vi "dfreq.vi"() -> ()   [LabVIEW 2019]
uses:
  <vilib>/DAQmx/read.llb/DAQmx Read (Counter DBL 1Chan 1Samp).vi
  <vilib>/DAQmx/create/channels.llb/DAQmx Create Channel (CO-Pulse Generation-Ticks).vi
  <vilib>/DAQmx/create/channels.llb/DAQmx Create Channel (CI-Frequency).vi
  <vilib>/DAQmx/configure/timing.llb/DAQmx Timing (Implicit).vi
  <vilib>/DAQmx/configure/trigger.llb/DAQmx Start Trigger (Digital Edge).vi
  <vilib>/DAQmx/miscellaneous.llb/DAQmx Fill In Error Info.vi
  <resource>/objmgr/daqmx.rc
panel:
  out "highest harmonic":i32
  out "counter":tag
  out "Array 2":dbl[](array[numeric])
  in  "stop":bool
  out "Array":tag[](array[tag])
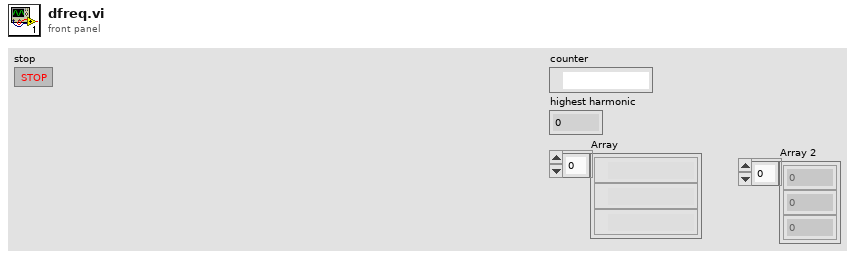
[diagram p1: front panel]
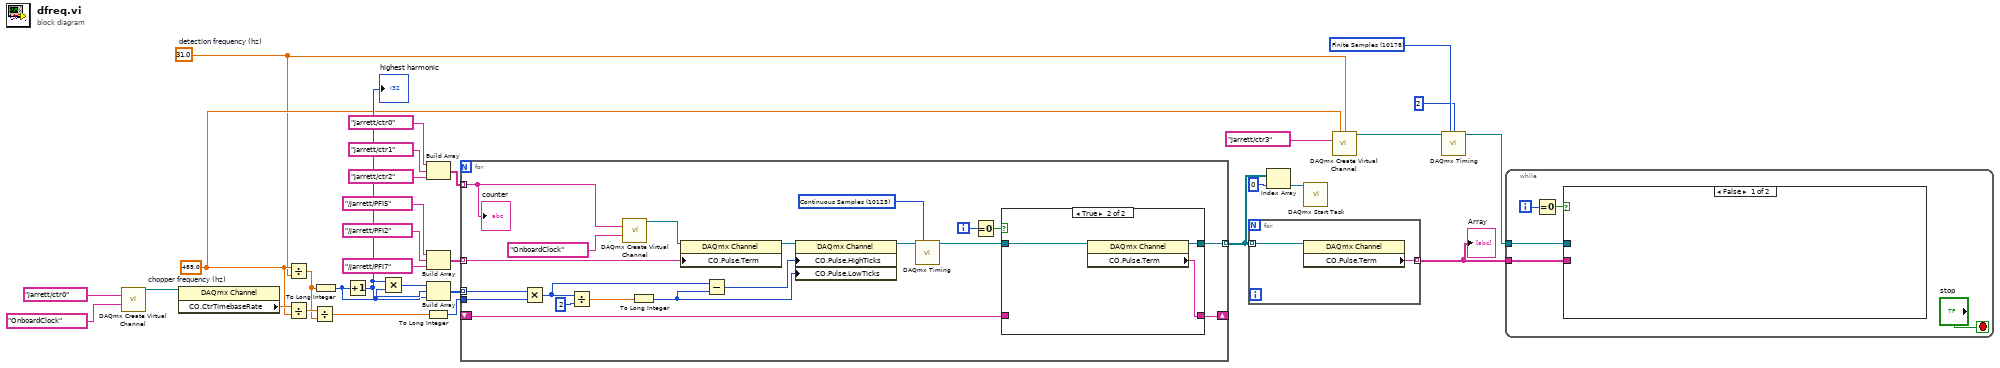
[diagram p0: block diagram]
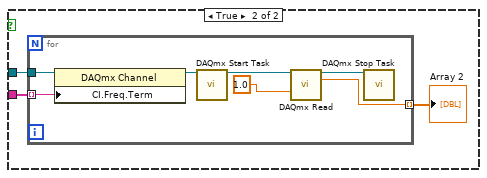
[diagram p2: hidden frame]
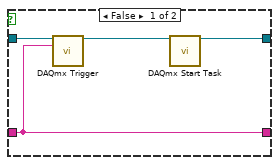
[diagram p3: hidden frame]
diagram:
  w11 = 10178 items=["Finite Samples"=10178, "Continuous Samples"=10123, "Hardware Timed Single Point"=12522] ("sample mode")
  w9 = 489.0  # chopper frequency (hz)
  w8 = 31.0  # detection frequency (hz)
  n1 = call-poly <vilib>:"DAQmx Create Virtual Channel.vi"("counter"=tag "jarrett/ctr0", "source of ticks"=tag "OnboardClock") -> ("task out"=w29:refnum<k21>)  [unwired: 12 in, 1 out]
  n2 = property class="DAQmx Channel"(reference=w29) -> ("CO.CtrTimebaseRate"=w28:dbl)  [unwired: 1 in, 2 out]
  n3 = Divide(x=w9, y=w8) -> (x/y=w25:dbl)
  n4 = Divide(x=w28, y=w9) -> (x/y=w27:dbl)
  n5 = Divide(x=w27, y=w25) -> (x/y=w26:dbl)
  n6 = To Long Integer(number=w25) -> (32bit integer=w19:i32)
  n7 = Increment(x=w19) -> (x+1=w20:i32)
  "highest harmonic" <- w20
  n8 = Multiply(x=w20, y=w19) -> (x*y=w21:i32)
  n9 = To Long Integer(number=w26) -> (32bit integer=w18:i32)
  n10 = Build Array(tag "jarrett/ctr0" ("counter"), tag "jarrett/ctr1" ("counter"), tag "jarrett/ctr2" ("counter")) -> (w23:tag[])
  n11 = Build Array(tag "/jarrett/PFI5" ("DAQmx Terminal"), tag "/jarrett/PFI2" ("DAQmx Terminal"), tag "/jarrett/PFI7" ("DAQmx Terminal")) -> (w1:tag[])
  n12 = Build Array(w21, w20, w19) -> (w22:i32[])
  n13 = for {
    tunnel: w23 -> [w50] mode=indexing
    tunnel: w22 -> [w45] mode=indexing
    tunnel: w18 -> [w46]
    tunnel: [w35] -> w15 mode=indexing
    shift-right: [w37] -> _
    shift-left: _ -> [w36]
    tunnel: w1 -> [w32] mode=indexing
    i -> [w40]
    w41 = 10123 items=["Finite Samples"=10178, "Continuous Samples"=10123, "Hardware Timed Single Point"=12522] ("sample mode")
    n14 = Multiply(x=w45, y=w46) -> (x*y=w47:i32)
    n15 = Divide(x=w47, y=2) -> (x/y=w48:dbl)
    n16 = call-poly <vilib>:"DAQmx Create Virtual Channel.vi"("counter"=w50, "source of ticks"=tag "OnboardClock") -> ("task out"=w34:refnum<k21>)  [unwired: 12 in, 1 out]
    n17 = To Long Integer(number=w48) -> (32bit integer=w44:i32)
    n18 = property class="DAQmx Channel"(reference=w34, "CO.Pulse.Term"=w32) -> (reference out=w33:refnum<k21>)  [unwired: 1 in, 1 out]
    n19 = Subtract(x=w47, y=w44) -> (x-y=w43:i32)
    n20 = property class="DAQmx Channel"(reference=w33, "CO.Pulse.HighTicks"=w43, "CO.Pulse.LowTicks"=w44) -> (reference out=w42:refnum<k21>)  [unwired: 1 in, 1 out]
    n21 = call-poly <vilib>:"DAQmx Timing.vi"("task/channels in"=w42, "sample mode"=w41) -> ("task out"=w38:refnum<k21>)  [unwired: 12 in, 1 out]
    n22 = Equal To 0?(x=w40) -> (x = 0?=w39:bool)
    n23 = case shown="True" w39 {
      tunnel: w38 -> [w54 w58]
      tunnel: [w55 w57] -> w37
      tunnel: w36 -> [w55 _]
      tunnel: [w52 w56] -> w35
      frame False {
        n24 = call-poly <vilib>:"DAQmx Trigger.vi"("task/channels in"=w54, "source"=w55) -> ("task out"=w53:refnum<k21>)  [unwired: 12 in, 1 out]
        n25 = call <vilib>:"DAQmx Start Task.vi"("task/channels in"=w53) -> ("task out"=w52:refnum<k21>)  [unwired: 13 in, 1 out]
      }
      frame True {
        n26 = property class="DAQmx Channel"(reference=w58) -> (reference out=w56:refnum<k21>, "CO.Pulse.Term"=w57:tag)  [unwired: 1 in, 1 out]
      }
    }
    "counter" <- w50
  }
  n27 = for {
    tunnel: w15 -> [w60] mode=indexing
    tunnel: [w59] -> w14 mode=indexing
    n28 = property class="DAQmx Channel"(reference=w60) -> ("CO.Pulse.Term"=w59:tag)  [unwired: 1 in, 2 out]
  }
  "Array" <- w14
  n29 = Index Array(array=w15, index=0) -> (element=w16:refnum<k21>)
  n30 = call <vilib>:"DAQmx Start Task.vi"("task/channels in"=w16) -> ()  [unwired: 13 in, 2 out]
  n31 = call-poly <vilib>:"DAQmx Create Virtual Channel.vi"("maximum value"=w9, "minimum value"=w8, "counter"=tag "jarrett/ctr3") -> ("task out"=w12:refnum<k21>)  [unwired: 11 in, 1 out]
  n32 = call-poly <vilib>:"DAQmx Timing.vi"("task/channels in"=w12, "sample mode"=w11, "samples per channel"=2) -> ("task out"=w7:refnum<k21>)  [unwired: 11 in, 1 out]
  n33 = while {
    tunnel: w14 -> [w65]
    tunnel: w7 -> [w63]
    i -> [w62]
    stop <- "stop" stop-if-true
    n34 = Equal To 0?(x=w62) -> (x = 0?=w61:bool)
    n35 = case shown="False" w61 {
      tunnel: w65 -> [_ w68]
      tunnel: w63 -> [_ w66]
      frame False {
      }
      frame True {
        n36 = for {
          tunnel: w68 -> [w71] mode=indexing
          tunnel: [w73] -> w67 mode=indexing
          tunnel: w66 -> [w69]
          n37 = property class="DAQmx Channel"(reference=w69, "CI.Freq.Term"=w71) -> (reference out=w75:refnum<k21>)  [unwired: 1 in, 1 out]
          n38 = call <vilib>:"DAQmx Start Task.vi"("task/channels in"=w75) -> ("task out"=w74:refnum<k21>)  [unwired: 13 in, 1 out]
          n39 = call-poly <vilib>:"DAQmx Read.vi"("task/channels in"=w74, "timeout"=1.0) -> ("task out"=w70:refnum<k21>, "data"=w73:dbl)  [unwired: 11 in, 1 out]
          n40 = call <vilib>:"DAQmx Stop Task.vi"("task/channels in"=w70) -> ()  [unwired: 13 in, 2 out]
        }
        "Array 2" <- w67
      }
    }
  }
